vi "Initialize.vi"(8 "error in":errorcluster, 11 "Plugin in":refnum<class "Tone Measurements.lvclass">) -> (0 "error out":errorcluster, 3 "Plugin out":refnum<class "Tone Measurements.lvclass">)   [LabVIEW 2025, in "Tone Measurements.lvlib" / "Tone Measurements.lvclass"]
uses:
  Tone Measurements.lvclass
  C:/Program Files/National Instruments/LabVIEW 2025/vi.lib/FlexLogger/SDK/PluginSDK.lvlibp/PEFClasses/SDK/Plugin/Plugin.lvclass
  <vilib>/FlexLogger/SDK/PluginSDK.lvlibp/PEFClasses/SDK/Processing Element/Timing Parameters.ctl
  <vilib>/FlexLogger/SDK/PluginSDK.lvlibp/PEFClasses/SDK/Processing Element/Timing Method.ctl
  <vilib>/FlexLogger/SDK/PluginSDK.lvlibp/PEFClasses/SDK/Producer Channel/Producer Channel.lvclass
  C:/Program Files/National Instruments/LabVIEW 2025/vi.lib/FlexLogger/SDK/PluginSDK.lvlibp/PEFClasses/SDK/Channel/Channel.lvclass
  <vilib>/FlexLogger/SDK/PluginSDK.lvlibp/PEFClasses/SDK/Plugin/ParameterAccess/Write Single Channel.vi
  <vilib>/FlexLogger/SDK/PluginSDK.lvlibp/PEFClasses/SDK/Plugin/ParameterAccess/Write DBL.vi
  <vilib>/FlexLogger/SDK/PluginSDK.lvlibp/PEFClasses/SDK/Plugin/ParameterAccess/Write I32.vi
  <vilib>/FlexLogger/SDK/PluginSDK.lvlibp/PEFClasses/SDK/Producer Channel/Create Producer Channel_v2.vi
  <vilib>/FlexLogger/SDK/PluginSDK.lvlibp/PEFClasses/SDK/Plugin/Plugin.lvclass
  C:/Program Files/National Instruments/LabVIEW 2025/vi.lib/FlexLogger/SDK/PluginSDK.lvlibp/PEFClasses/SDK/Processing Element/Processing Element.lvclass
  C:/dev/dsb/niflexlogger-plugins/PDK plugins/Tone Measurements/source/Tone Measurements.lvclass
  <vilib>/FlexLogger/SDK/PluginSDK.lvlibp
  <vilib>/FlexLogger/SDK/PluginSDK.lvlibp/PEFClasses/SDK/Processing Element/Processing Element.lvclass
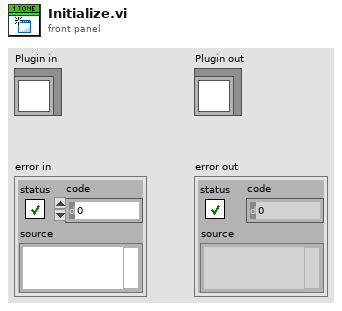
[diagram p1: front panel]
types:
  T1 = typedef "PluginSDK.lvlibp/Processing Element.lvclass/Timing Parameters.ctl" = cluster{"Timing Method":T2, "Timing Period (ms)":i32}
  T2 = typedef "PluginSDK.lvlibp/Processing Element.lvclass/Timing Method.ctl" = enum16{"Periodic", "Immediate", "On Data Ready", "Triggered"}
  T3 = cluster{"Unique Channel Identifier":string, "Long Name":string, "Unit":string}[]
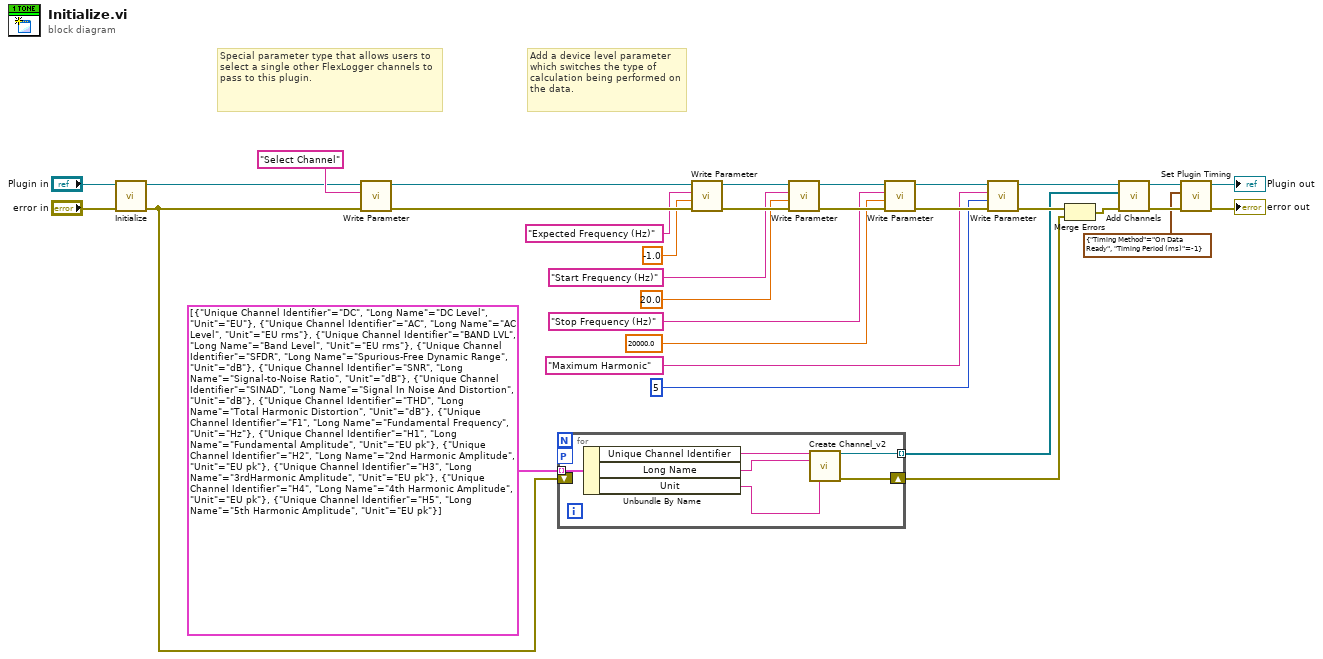
[diagram p0: block diagram]
diagram:
  # "Add a device level parameter which switches the type of calculation being performed on the data."
  # "Special parameter type that allows users to select a single other FlexLogger channels to pass to this plugin."
  n1 = call-parent "Initialize.vi"("error in (no error)"="error in", "Plugin in"="Plugin in") -> ("error out"=w7:errorcluster, "Plugin out"=w26:refnum<class "Tone Measurements.lvclass">)  [unwired: 8 in]
  n2 = call-poly <vilib>:"Write Parameter.vi"("error in (no error)"=w7, "Name (Unique Channel Identifier)"="Select Channel" ("Name"), "Plugin in"=w26) -> ("error out"=w28:errorcluster, "Plugin out"=w29:refnum<class "Tone Measurements.lvclass">)  [unwired: 7 in]
  n3 = for {
    tunnel: T3 [{"Unique Channel Identifier"="DC", "Long Name"="DC Level", "Unit"="EU"}, {"Unique Channel Identifier"="AC", "Long Name"="AC Level", "Unit"="EU rms"}, {"Unique Channel Identifier"="BAND LVL", "Long Name"="Band Level", "Unit"="EU rms"}, {"Unique Channel Identifier"="SFDR", "Long Name"="Spurious-Free Dynamic Range", "Unit"="dB"}, {"Unique Channel Identifier"="SNR", "Long Name"="Signal-to-Noise Ratio", "Unit"="dB"}, {"Unique Channel Identifier"="SINAD", "Long Name"="Signal In Noise And Distortion", "Unit"="dB"}, {"Unique Channel Identifier"="THD", "Long Name"="Total Harmonic Distortion", "Unit"="dB"}, {"Unique Channel Identifier"="F1", "Long Name"="Fundamental Frequency", "Unit"="Hz"}, {"Unique Channel Identifier"="H1", "Long Name"="Fundamental Amplitude", "Unit"="EU pk"}, {"Unique Channel Identifier"="H2", "Long Name"="2nd Harmonic Amplitude", "Unit"="EU pk"}, {"Unique Channel Identifier"="H3", "Long Name"="3rdHarmonic Amplitude", "Unit"="EU pk"}, {"Unique Channel Identifier"="H4", "Long Name"="4th Harmonic Amplitude", "Unit"="EU pk"}, {"Unique Channel Identifier"="H5", "Long Name"="5th Harmonic Amplitude", "Unit"="EU pk"}] -> [w38] mode=indexing
    tunnel: [w34] -> w8 mode=indexing
    workers-P: _ -> [_]
    shift-right: [w33] -> w6
    shift-left: w7 -> [_]
    n4 = Unbundle By Name(w38) -> ("Unique Channel Identifier"=w37:string, "Long Name"=w36:string, "Unit"=w35:string)
    n5 = call-poly <vilib>:"Create Channel_v2.vi"("Unique Channel Identifier"=w37, "Default Channel Name"=w36, "Unit"=w35) -> ("Producer Channel"=w34:refnum<class "Producer Channel.lvclass">, "error out"=w33:errorcluster)  [unwired: 11 in]
  }
  n6 = call-poly <vilib>:"Write Parameter.vi"("error in (no error)"=w28, "Value"=-1.0, "Name"="Expected Frequency (Hz)", "Plugin in"=w29) -> ("error out"=w23:errorcluster, "Plugin out"=w24:refnum<class "Tone Measurements.lvclass">)  [unwired: 6 in]
  n7 = call-poly <vilib>:"Write Parameter.vi"("error in (no error)"=w23, "Value"=20.0, "Name"="Start Frequency (Hz)", "Plugin in"=w24) -> ("error out"=w22:errorcluster, "Plugin out"=w21:refnum<class "Tone Measurements.lvclass">)  [unwired: 6 in]
  n8 = call-poly <vilib>:"Write Parameter.vi"("error in (no error)"=w22, "Value"=20000.0, "Name"="Stop Frequency (Hz)", "Plugin in"=w21) -> ("error out"=w20:errorcluster, "Plugin out"=w19:refnum<class "Tone Measurements.lvclass">)  [unwired: 6 in]
  n9 = call-poly <vilib>:"Write Parameter.vi"("error in (no error)"=w20, "Value"=5, "Name"="Maximum Harmonic", "Plugin in"=w19) -> ("error out"=w11:errorcluster, "Plugin out"=w18:refnum<class "Tone Measurements.lvclass">)  [unwired: 6 in]
  n10 = Merge Errors(w11, w6) -> (w10:errorcluster)
  n11 = call <vilib>:"Add Channels.vi"("error in (no error)"=w10, "Channels"=w8, "Plugin in"=w18) -> ("error out"=w5:errorcluster, "Plugin out"=w3:refnum<class "Tone Measurements.lvclass">)  [unwired: 7 in]
  n12 = call <vilib>:"Set Plugin Timing.vi"("error in (no error)"=w5, "Timing Parameters"=T1 {"Timing Method"=enum."On Data Ready", "Timing Period (ms)"=-1}, "Plugin in"=w3) -> ("error out"=→"error out":errorcluster, "Plugin out"=→"Plugin out":refnum<class "Tone Measurements.lvclass">)  [unwired: 7 in]
